vi "set LTE BW and DL Channel Number.vi"(8 "error in (no error)":errorcluster caption="에러 입력(에러 없음)", 9 "PCC Downlink":i32, 10 "BandWidth":T1, 11 "Anritsu Call Box_Implement 입력":refnum<class "Anritsu Call Box_Implement.lvclass">) -> (0 "error out":errorcluster caption="에러 출력", 3 "Anritsu Call Box_Implement 출력":refnum<class "Anritsu Call Box_Implement.lvclass">)   [LabVIEW 2023, in "ANRITSU Call Box.lvlib" / "Anritsu Call Box_Implement.lvclass"]
uses:
  Anritsu Call Box_Implement.lvclass
  Anritsu Call Box_Implement.lvclass/Anritsu Call Box_Implement.ctl
  LTE/LTE.lvclass
  Type Definition/LTE Supported BandWidth.ctl
  ANRITSU Call Box.lvlib
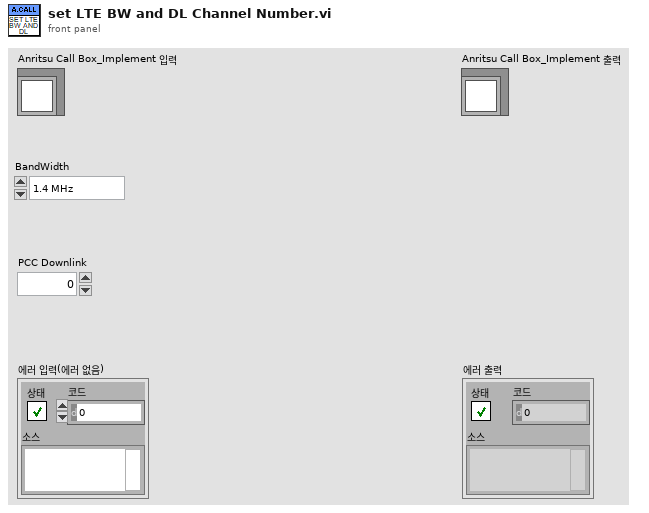
[diagram p1: front panel]
types:
  T1 = typedef "ANRITSU Call Box.lvlib/LTE Supported BandWidth.ctl" = enum16{"1.4 MHz", "3 MHz", "5 MHz", "10 MHz", "15 MHz", "20 MHz"}
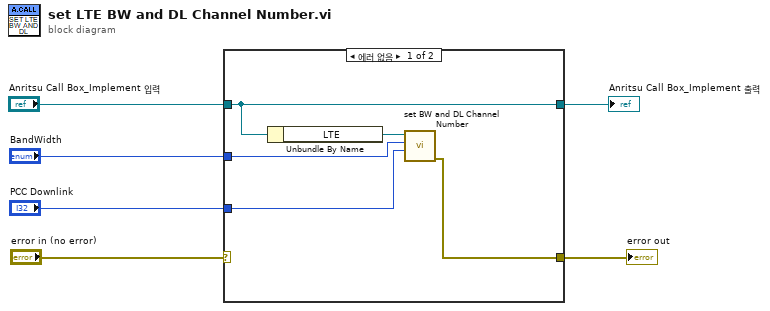
[diagram p0: block diagram]
diagram:
  n1 = case shown="에러 없음" "error in (no error)" {
    selector: "error in (no error)" -> [_ w12]
    tunnel: "Anritsu Call Box_Implement 입력" -> [w11 w13]
    tunnel: [w11 w13] -> w5
    tunnel: [w7 w12] -> w3
    tunnel: "BandWidth" -> [w9 _]
    tunnel: "PCC Downlink" -> [w8 _]
    frame No Error {
      n2 = Unbundle By Name(w11) -> ("LTE"=w10:refnum<class "LTE.lvclass">)
      n3 = call "set BW and DL Channel Number.vi"("PCC Downlink"=w8, "BandWidth"=w9, "LTE 입력"=w10) -> ("error out"=w7:errorcluster)  [unwired: 7 in, 1 out]
    }
    frame Error {
    }
  }
  "error out" <- w3
  "Anritsu Call Box_Implement 출력" <- w5
